vi "Delete Scripting API.vi"(11 "Arguments":string[](array[string])) -> (2 "Output/Failure Message":string, 3 "Exit Code":i32)   [LabVIEW 2019, in "Build VIs.lvlib"]
uses:
  Build VIs.lvlib
panel:
  out "error out":errorcluster
  in  "error in":errorcluster
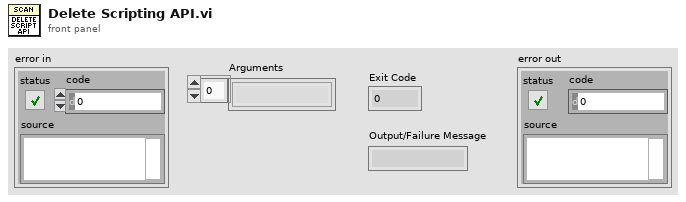
[diagram p1: front panel]
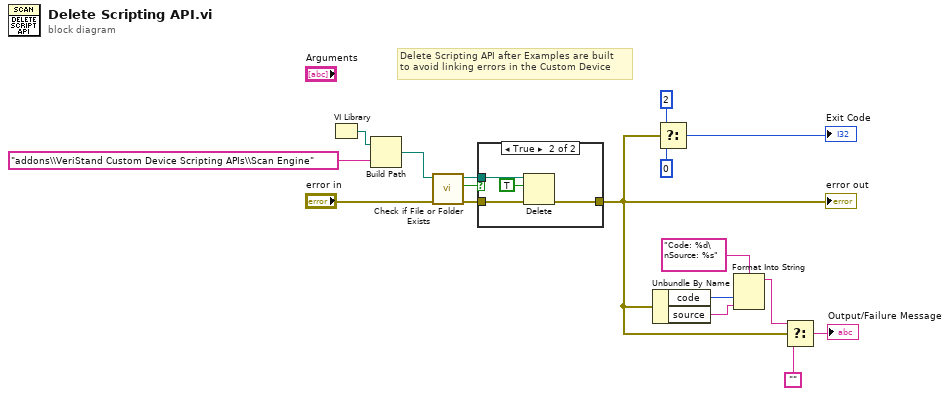
[diagram p0: block diagram]
diagram:
  # "Delete Scripting API after Examples are built\nto avoid linking errors in the Custom Device"
  n1 = VI Library() -> (path=w13:path)
  n2 = Build Path(base path=w13, name or relative path="addons\\VeriStand Custom Device Scripting APIs\\Scan Engine") -> (appended path=w14:path)
  n3 = call <vilib>:"Check if File or Folder Exists.vi"("error in (no error)"="error in", "path"=w14) -> ("error out"=w15:errorcluster, "file or folder exists?"=w17:bool, "dup path"=w16:path)  [unwired: 7 in]
  n4 = case shown="True" w17 {
    tunnel: w16 -> [_ w22]
    tunnel: w15 -> [w18 w20]
    tunnel: [w18 w19] -> w3
    frame False {
    }
    frame True {
      n5 = Delete(path (use dialog)=w22, entire hierarchy (F)=TRUE, error in=w20) -> (error out=w19:errorcluster)  [unwired: 2 in, 2 out]
    }
  }
  "error out" <- w3
  n6 = Unbundle By Name(w3) -> ("code"=w10:i32, "source"=w9:string)
  n7 = Select(t=2 ("Exit Code"), s=w3, f=0 ("Exit Code")) -> (s? t:f=→"Exit Code":i32)
  n8 = Format Into String(format string="Code: %d\nSource: %s", w10, w9) -> (resulting string=w8:string)  [unwired: 2 in, 1 out]
  n9 = Select(t=w8, s=w3, f="") -> (s? t:f=→"Output/Failure Message":string)
